vi "Compteurs + Debit.vi"() -> ()   [LabVIEW 2022 SP3]
uses:
  <vilib>/Platform/TimedLoop/XDataNode/timing_clust.ctl
  <vilib>/Platform/TimedLoop/XDataNode/nitl_modes.ctl
  <vilib>/Platform/TimedLoop/XDataNode/wakeup.ctl
  Variables globales/Variable glob generale.vi
  Variables globales/Variable globale compteurs.vi
  <vilib>/Platform/TimedLoop/XDataNode/XDataNode.xnode
  <vilib>/Platform/TimedLoop/XDataNode/XDNodeRunTimeDep.lvlib
  <vilib>/Utility/config.llb/NI_LVConfig.lvlib
panel:
  out "Temps débit":u16
  out "data+débit compteur":string[][](array[string])
  # "acquisition data compteur\net calcul débit"
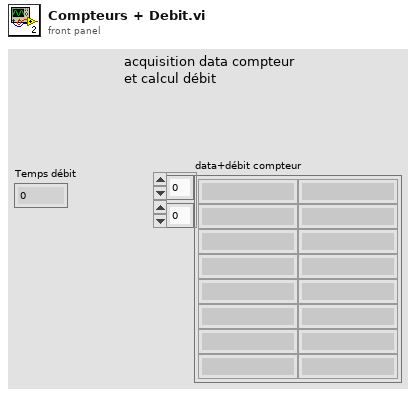
[diagram p1: front panel]
types:
  T1 = typedef "XDNodeRunTimeDep.lvlib/timing_clust.ctl" = cluster{"Expected End [f-1]":u64, "Actual End [f-1]":u64, "Finished Late? [f-1]":bool, "Expected End [i-1]":u64, "Actual End [i-1]":u64, "Finished Late? [i-1]":bool, "Expected Start [i]":u64, "Actual Start [i]":u64, "Expected Start [f]":u64, "Actual Start [f]":u64, "Source Name":string, "Structure Name":string, "Period":i64, "Deadline":i64, "Offset":i64, "Start":i64, "Priority":i32, "Timeout":i32, "Mode":T2, "Wakeup Reason":T3, "Error":errorcluster, "Source Type":string, "Secondary Source Type":string, "Global End Time":u64, "Global Start Time":u64, "Frame Duration":u64, "Iteration Duration":u64, "Assigned CPU":i32, "I/O Scan Engine Mode":u32}
  T2 = typedef "XDNodeRunTimeDep.lvlib/nitl_modes.ctl" = enum32{"No Change", "Process missed periods, maintain original phase", "Discard missed periods, maintain original phase", "Process missed periods, ignore original phase", "Discard missed periods, ignore original phase"}
  T3 = typedef "XDNodeRunTimeDep.lvlib/wakeup.ctl" = enum32{"Normal", "Aborted", "Asynchronous wakeup", "Timing source error", "Timed loop error", "Timeout"}
  T4 = enum32{"Bad", "Idle", "Run top level", "Running"}
  T5 = cluster{"Nom tache compteurs":refnum<k21>, "Noms des compteurs":string[], "Selection":bool[], "Init compteurs":dbl[], "Noms compteurs selectionnes":string[]}
  T6 = typedef "NI_LVConfig.lvlib/Config Data RefNum.ctl" = refnum<k1>
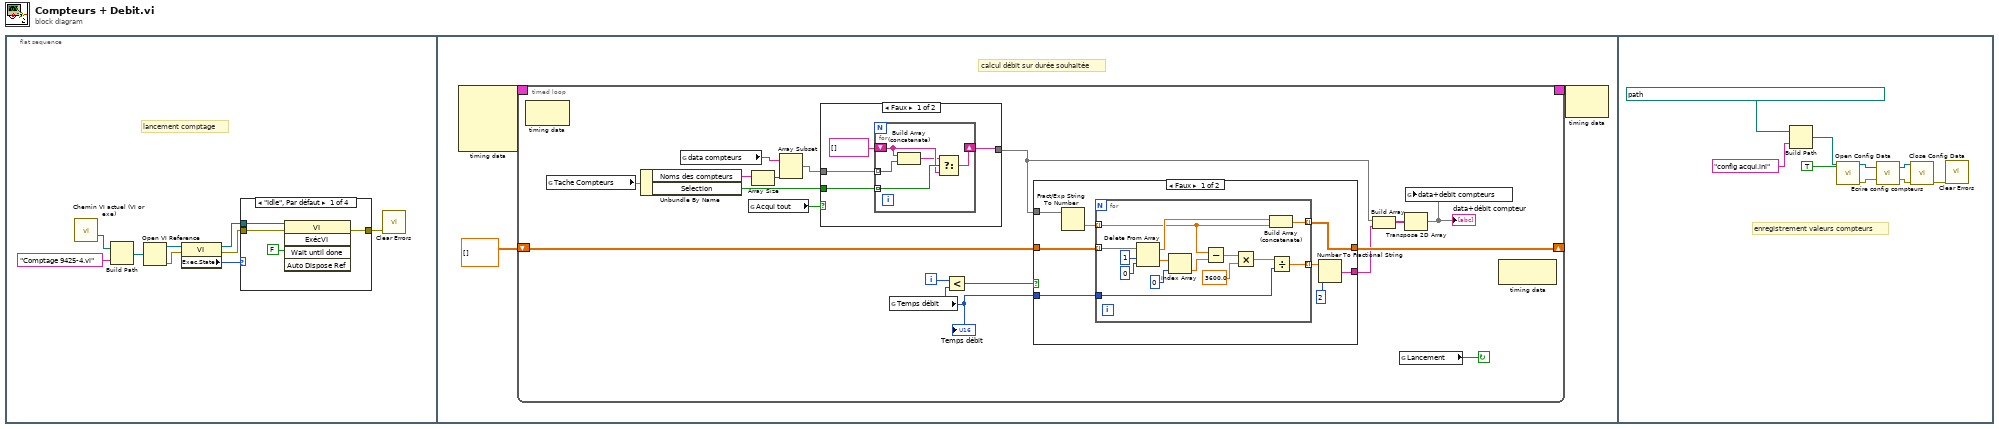
[diagram p0: block diagram]
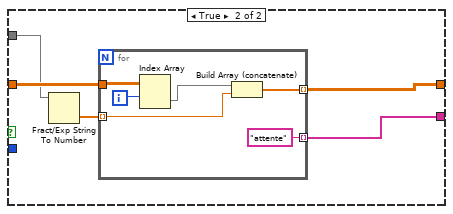
[diagram p6: hidden frame]
diagram:
  n1 = flat-sequence {
    frame #0 {
      # "lancement comptage"
      n2 = call "Chemin VI actuel (VI or exe).vi"() -> ("VI or executable installation directory"=w1:path)  [unwired: 14 in, 1 out]
      n3 = Build Path(base path=w1, name or relative path="Comptage 9425-4.vi" ("nom ou chemin relatif")) -> (appended path=w8:path)
      n4 = Open VI Reference(vi path=w8) -> (vi reference=w3:refnum<vi>, error out=w4:errorcluster)  [unwired: 5 in]
      n5 = property class="VI"(reference=w3, error in=w4) -> (reference out=w6:refnum<vi>, error out=w5:errorcluster, "Exec.State"=w7:T4)
      n6 = case shown="\"Idle\", Par défaut" w7 {
        tunnel: w6 -> [w12 _ _ _]
        tunnel: w5 -> [w11 w14 w15 w16]
        tunnel: [w10 w14 w15 w16] -> w2
        frame "Idle", Default {
          n7 = invoke class="VI" method="ExécVI"(reference=w12, error in=w11, "Wait until done"=FALSE ("Attendre la fin")) -> (error out=w10:errorcluster)  [unwired: 2 in, 4 out]
        }
        frame "Run top level" {
        }
        frame "Running" {
        }
        frame "Bad" {
        }
      }
      n8 = call <vilib>:"Clear Errors.vi"("error in (no error)"=w2) -> ()  [unwired: 5 in, 2 out]
    }
    frame #1 {
      # "calcul débit sur durée souhaitée"
      n9 = node-c288() -> (w19:T1)  [unwired: 4 in]
      n10 = timed-loop {
        timing: w19 -> [_]
        timing-out: [_] -> w18
        shift-right: [w34] -> _
        shift-left: dbl[][] [] -> [w35]
        i -> [w33]
        stop <- w36 continue-if-true
        n11 = node-c288() -> ()  [unwired: 1 in, 1 out]
        n12 = global read "Variable globale compteurs.vi" "Tache Compteurs"() -> (w27:T5)
        n13 = Unbundle By Name(w27) -> ("Noms des compteurs"=w23:string[], "Selection"=w24:bool[])
        n14 = global read "Variable globale compteurs.vi" "data compteurs"() -> (w26:string[])
        n15 = global read "Variable glob generale.vi" "Acqui tout"() -> (w21:bool)
        n16 = Array Size(array=w23) -> (size(s)=w25:i32)
        n17 = Array Subset(array=w26, length=w25) -> (w22:string[])  [unwired: 1 in]
        n18 = case shown="Faux" w21 {
          tunnel: w24 -> [w40 _]
          tunnel: w22 -> [w39 w46]
          tunnel: [w37 w46] -> w20
          frame False {
            n19 = for {
              tunnel: w40 -> [w45] mode=indexing
              tunnel: w39 -> [w42] mode=indexing
              shift-right: [w44] -> w37
              shift-left: string[] [] -> [w43]
              n20 = Build Array (concatenate)(w43, w42) -> (w41:string[])
              n21 = Select(t=w41, s=w45, f=w43) -> (s? t:f=w44:string[])
            }
          }
          frame True {
          }
        }
        n22 = global read "Variable globale compteurs.vi" "Temps débit"() -> (w31:u16)
        "Temps débit" <- w31
        n23 = Less?(x=w33, y=w31) -> (x < y?=w32:bool)
        n24 = case shown="Faux" w32 {
          tunnel: w35 -> [w54 w73]
          tunnel: [w53 w72] -> w34
          tunnel: w31 -> [w51 _]
          tunnel: w20 -> [w48 w70]
          tunnel: [w47 w69] -> w30
          frame False {
            n25 = Fract/Exp String To Number(string=w48) -> (number=w52:dbl[])  [unwired: 3 in, 1 out]
            n26 = for {
              tunnel: w52 -> [w61] mode=indexing
              tunnel: w54 -> [w68] mode=indexing
              tunnel: [w64] -> w53 mode=indexing
              tunnel: w51 -> [w56]
              tunnel: [w55] -> w50 mode=indexing
              n27 = Delete From Array(array=w68, length=1 ("longueur"), index=0 ("indice")) -> (deleted portion=w63:dbl[], array with subset deleted=w65:dbl[])
              n28 = Index Array(array=w63, index=0 ("indice")) -> (element=w60:dbl)
              n29 = Subtract(x=w61, y=w60) -> (x-y=w59:dbl)
              n30 = Multiply(x=w59, y=3600.0) -> (x*y=w57:dbl)
              n31 = Build Array (concatenate)(w65, w61) -> (w64:dbl[])
              n32 = Divide(x=w57, y=w56) -> (x/y=w55:dbl)
            }
            n33 = Number To Fractional String(number=w50, precision (6)=i16 2 ("précision (6)")) -> (F-format string=w47:string[])  [unwired: 2 in]
          }
          frame True {
            n34 = Fract/Exp String To Number(string=w70) -> (number=w71:dbl[])  [unwired: 3 in, 1 out]
            n35 = for {
              tunnel: w71 -> [w79] mode=indexing
              tunnel: w73 -> [w76]
              tunnel: [w78] -> w72 mode=indexing
              tunnel: ["attente"] -> w69 mode=indexing
              i -> [w75]
              n36 = Index Array(array=w76, index (row)=w75) -> (element=w74:dbl[])  [unwired: 1 in]
              n37 = Build Array (concatenate)(w74, w79) -> (w78:dbl[])
            }
          }
        }
        n38 = Build Array(w20, w30) -> (w29:string[][])
        n39 = global read "Variable glob generale.vi" "Lancement"() -> (w36:bool)
        n40 = Transpose 2D Array(2D array=w29) -> (transposed array=w28:string[][])
        "data+débit compteur" <- w28
        n41 = global write "Variable globale compteurs.vi" "data+debit compteurs"(w28) -> ()
        n42 = node-c288() -> ()  [unwired: 1 in, 1 out]
      }
      n43 = node-c288(w18) -> ()  [unwired: 1 out]
    }
    frame #2 {
      # "enregistrement valeurs compteurs"
      n44 = Build Path(base path=path "C:/LABVIEW/PRES+TEMP+REG dernière version/Configurations", name or relative path="config acqui.ini" ("nom ou chemin relatif")) -> (appended path=w90:path)
      n45 = call <vilib>:"Open Config Data.vi"("create file if necessary (T)"=TRUE ("create file if necessary? (T)"), "configuration file path"=w90) -> ("error out"=w87:errorcluster, "refnum"=w88:T6)  [unwired: 7 in, 1 out]
      n46 = call "Ecrire config compteurs.vi"("error in (no error)"=w87, "refnum"=w88) -> ("error out"=w84:errorcluster, "refnum out"=w85:T6)
      n47 = call <vilib>:"Close Config Data.vi"("error in (no error)"=w84, "refnum"=w85) -> ("error out"=w86:errorcluster)  [unwired: 8 in, 1 out]
      n48 = call <vilib>:"Clear Errors.vi"("error in (no error)"=w86) -> ()  [unwired: 5 in, 2 out]
    }
  }
